vi "UE_Cycles_Done.vi"(1 "requested":i32, 2 "completed":i32) -> (0 "done":bool)   [LabVIEW 2026]
doc: "INTENT: Check whether completed cycles meet requested number. INPUTS: completed (int32), requested (int32). OUTPUTS: done (bool). DESIGN CONSTRAINT: Counter persistence and retry identities are managed by Cycle Manager. REQUIREMENTS: SRS-F-010. No physical hardware side effects. Acceptance requires native LabVIEW compilation and behavioral testing."
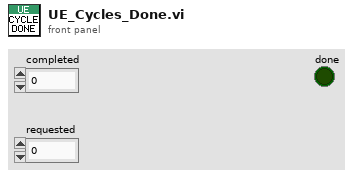
[diagram p1: front panel]
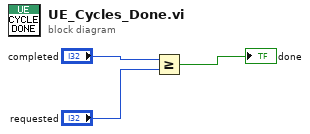
[diagram p0: block diagram]
diagram:
  n1 = Greater Or Equal?(x="completed", y="requested") -> (x >= y?=→"done":bool)
